vi "Get_Input.vi"(8 "error in (no error)":errorcluster, 11 "object in":refnum<class "AIO_Channel.lvclass">) -> (0 "error out":errorcluster, 2 "Input":dbl, 3 "object out":refnum<class "AIO_Channel.lvclass">)   [LabVIEW 2021, in "Simulator-Channel.lvlib" / "AIO_Channel.lvclass"]
doc: "Gets the Input"
uses:
  AIO_Channel.lvclass
  C:/Users/averna/Documents/LV Gym DEMO/Factory Pattern/Device Channels/Dependencies/AIO-Channel.lvlibp/Channels/AIO-Channel/AIO_Channel_class/AIO_Channel.lvclass
  AIO_Channel.lvclass/AIO_Channel.ctl
  AIO_Panel/DIO_Panel Messages/Get Input Msg/Get Input Msg.lvclass/Get Input Msg.ctl
  <vilib>/ActorFramework/Message Enqueuer/Message Enqueuer.lvclass/Message Enqueuer.ctl
  <vilib>/ActorFramework/Message Enqueuer/Enqueue.vi
  AIO_Panel/DIO_Panel Messages/Get Input Msg/Get Input Msg.lvclass
  C:/Program Files/National Instruments/LabVIEW 2021/vi.lib/ActorFramework/Message/Message.lvclass
  Dependencies/AIO-Channel.lvlibp/Channels/AIO-Channel/AIO_Channel_class/Properties/GetAIOConfiguration.vi
  <vilib>/ActorFramework/Message Priority Queue/Priority Enqueue.vi
  Dependencies/AIO-Channel.lvlibp/Channels/AIO-Channel/AIO-Configuration_class/AIO-Configuration.lvclass
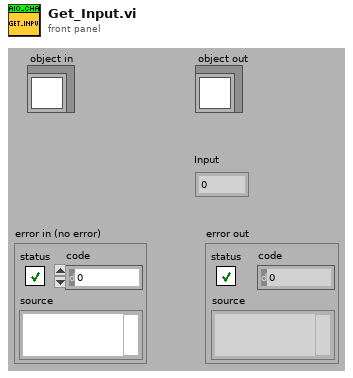
[diagram p1: front panel]
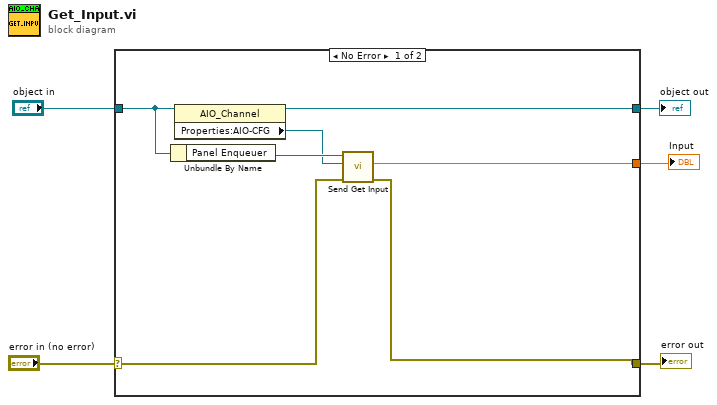
[diagram p0: block diagram]
diagram:
  n1 = case shown="No Error" "error in (no error)" {
    selector: "error in (no error)" -> [w8 w14]
    tunnel: [w7 w14] -> w4
    tunnel: [w10 w13] -> w2
    tunnel: "object in" -> [w12 w13]
    tunnel: [w6 _] -> w1
    frame No Error {
      n2 = Unbundle By Name(w12) -> ("Panel Enqueuer"=w11:refnum<class "Message Enqueuer.lvclass">)
      n3 = property class="AIO_Channel"(reference=w12) -> (reference out=w10:refnum<class "AIO_Channel.lvclass">, "Properties:AIO-CFG"=w9:refnum<class "AIO-Configuration.lvclass">)  [unwired: 1 in, 1 out]
      n4 = call "Send Get Input.vi"("error in (no error)"=w8, "AIO_CFG"=w9, "Message Enqueuer"=w11) -> ("error out"=w7:errorcluster, "Input"=w6:dbl)  [unwired: 6 in, 1 out]
    }
    frame Error {
    }
  }
  "error out" <- w4
  "object out" <- w2
  "Input" <- w1
